vi "Add Item.vi"(7 "Action":T1, 8 "error in (no error)":errorcluster, 11 "Listbox Refs in":T2 {"Section Ref" format="%.0x"}) -> (0 "error out":errorcluster, 3 "Listbox Refs out":T2 {"Section Ref" format="%.0x"})   [LabVIEW 2019, in "FPGA Addon System Explorer.lvlib"]
uses:
  FPGA Addon System Explorer.lvlib
  Types/Listbox Cluster.ctl
  <vilib>/NI VeriStand/Custom Device API/Custom Device Item Ref.ctl
  Types/Channel Type.ctl
  Addon Shared/Types/FG Action.ctl
  <vilib>/NI VeriStand/Custom Device API/Custom Device Channel.ctl
  <vilib>/NI VeriStand/Custom Device API/Custom Device Channel Type.ctl
  Addon Shared/SubVIs/Constants.vi
  <vilib>/NI/NI VeriStand Advanced SysDef API/SysDef API/SysDef.Property.Get.vi
  <vilib>/NI/NI VeriStand Advanced SysDef API/_SubVIs/SysDef.Property.Get.Variant.vi
  <vilib>/NI/NI VeriStand Advanced SysDef API/SysDef API/SysDef.Property.Set.vi
  <vilib>/NI/NI VeriStand Advanced SysDef API/_SubVIs/SysDef.Property.Set.Variant.vi
  <vilib>/NI VeriStand/Custom Device API/Custom Device API.lvlib
  Addon Shared/FPGA Addon Shared.lvlib
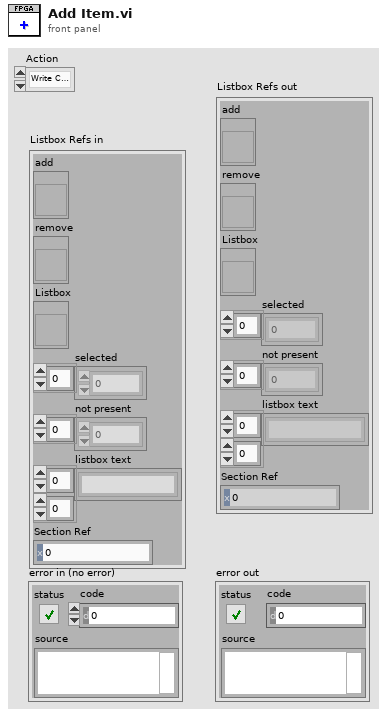
[diagram p1: front panel]
types:
  T1 = typedef "FPGA Addon System Explorer.lvlib/Channel Type.ctl" = enum16{"Write Channel", "Read Channel", "Write Waveform", "Read Waveform"}
  T2 = typedef "FPGA Addon System Explorer.lvlib/Listbox Cluster.ctl" = cluster{"add":refnum<vi>, "remove":refnum<vi>, "Listbox":refnum<vi>, "selected":i32[], "not present":i32[], "listbox text":string[][], "Section Ref":T3}
  T3 = typedef "Custom Device API.lvlib/Custom Device Item Ref.ctl" = u64
  T4 = typedef "FPGA Addon Shared.lvlib/FG Action.ctl" = enum8{"GET", "SET"}
  T5 = typedef "FPGA Addon Shared.lvlib/Register Information.ctl" = cluster{"Name":string, "Data Type":T6, "Default Value":variant}
  T6 = typedef "FPGA Addon Shared.lvlib/Data Type.ctl" = enum8{"<Null>", "I8", "I16", "I32", "I64", "U8", "U16", "U32", "U64", "SGL", "Boolean", "Analog PWM In Settings", "Analog PWM In", "Digital PWM In Settings", "Digital PWM In", "Digital PWM Out", "Sine Out", "FXP+/-24.5", "FXP+/-16.5", "FXP+/-32.8", "FXP+/-64.32", "FXP+/-16.7", "FXP+/-20.5", "FXP+/-27.5", "FXP+/-32.16", "FXP+16.3", "FXP+18.3", "Digital Static In", "Digital Static Out", "Digital Static In Settings", "Digital WSS Out", "Quad Encoder Settings", "Quad Encoder In", "Group"}
  T7 = typedef "Custom Device API.lvlib/Custom Device Channel.ctl" = cluster{"Type":T8, "Units":string, "Default Value":dbl, "Faultable":bool, "Scalable":bool}
  T8 = typedef "Custom Device API.lvlib/Custom Device Channel Type.ctl" = enum16{"Input", "Output"}
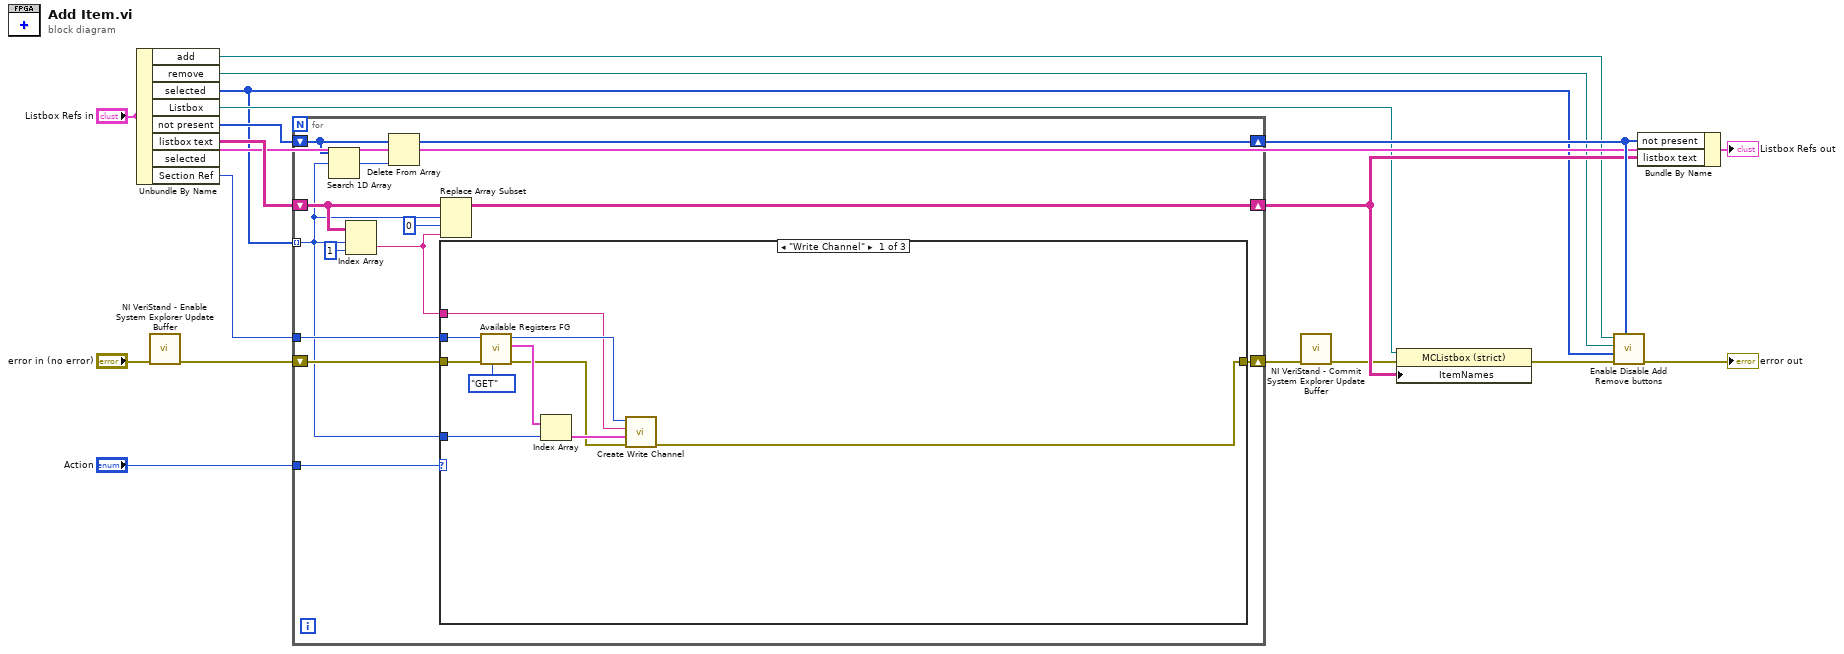
[diagram p0: block diagram]
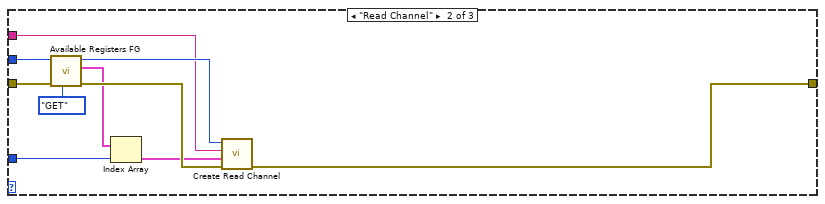
[diagram p2: hidden frame]
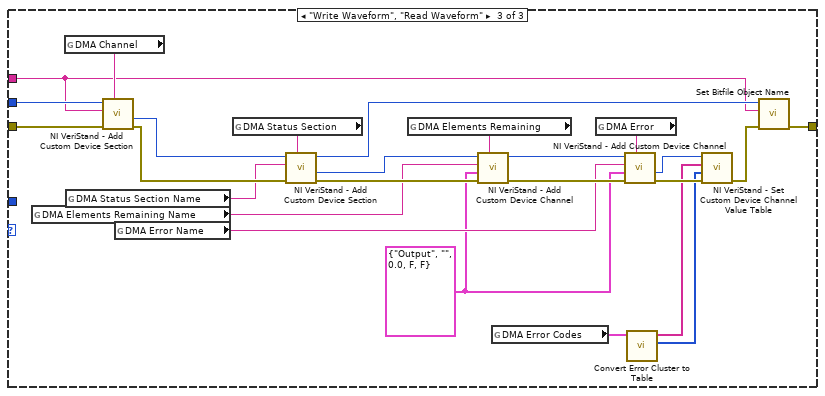
[diagram p3: hidden frame]
diagram:
  n1 = Unbundle By Name("Listbox Refs in") -> ("add"=w10:refnum<vi>, "remove"=w11:refnum<vi>, "selected"=w3:i32[], "Listbox"=w4:refnum<vi>, "not present"=w9:i32[], "listbox text"=w17:string[][], "Section Ref"=w5:T3)  [unwired: 1 out]
  n2 = call <vilib>:"NI VeriStand - Enable System Explorer Update Buffer.vi"("error in (no error)"="error in (no error)") -> ("error out"=w8:errorcluster)  [unwired: 10 in]
  n3 = for {
    tunnel: w5 -> [w30]
    shift-right: [w19] -> w6
    shift-left: w8 -> [w31]
    tunnel: w3 -> [w21] mode=indexing
    shift-right: [w27] -> w15
    shift-left: w17 -> [w28]
    shift-right: [w23] -> w16
    shift-left: w9 -> [w25]
    tunnel: "Action" -> [w22]
    n4 = Search 1D Array(1D array=w25, element=w21) -> (index of element=w24:i32)  [unwired: 1 in]
    n5 = Index Array(array=w28, index (row)=w21, index (col)=1 ("disabled index (col)")) -> (element=w20:string)
    n6 = Delete From Array(array=w25, index=w24) -> (array with subset deleted=w23:i32[])  [unwired: 1 in, 1 out]
    n7 = case shown="\"Write Channel\"" w22 {
      tunnel: w31 -> [w38 w48 w75]
      tunnel: [w34 w51 w53] -> w19
      tunnel: w30 -> [w37 w49 w76]
      tunnel: w20 -> [w32 w42 w52]
      tunnel: w21 -> [w35 w45 _]
      frame "Write Channel" {
        n8 = call "Available Registers FG.vi"("Action"=FG_Action."GET", "error in (no error)"=w38, "Item Ref"=w37) -> ("error out"=w36:errorcluster, "Available Registers"=w40:T5[], "Item Ref out"=w33:T3)  [unwired: 6 in]
        n9 = Index Array(array=w40, index=w35) -> (element=w39:T5)
        n10 = call "Create Write Channel.vi"("error in (no error)"=w36, "Cluster"=w39, "Bitfile Name"=w32, "Item Ref in"=w33) -> ("error out"=w34:errorcluster)  [unwired: 7 in]
      }
      frame "Read Channel" {
        n11 = call "Available Registers FG.vi"("Action"=FG_Action."GET", "error in (no error)"=w48, "Item Ref"=w49) -> ("error out"=w47:errorcluster, "Available Registers"=w46:T5[], "Item Ref out"=w43:T3)  [unwired: 6 in]
        n12 = Index Array(array=w46, index=w45) -> (element=w44:T5)
        n13 = call "Create Read Channel.vi"("error in (no error)"=w47, "Channel"=w44, "Bitfile Name"=w42, "Item Ref in"=w43) -> ("error out"=w51:errorcluster)  [unwired: 7 in]
      }
      frame "Write Waveform", "Read Waveform" {
        w63 = T7 {"Type"=enum."Output", "Units"="", "Default Value"=0.0, "Faultable"=FALSE, "Scalable"=FALSE} ("Channel")
        n14 = global read "Constants.vi" "DMA Elements Remaining Name"() -> (w66:string)
        n15 = global read "Constants.vi" "DMA Channel"() -> (w74:string)
        n16 = global read "Constants.vi" "DMA Status Section Name"() -> (w62:string)
        n17 = call <vilib>:"NI VeriStand - Add Custom Device Section.vi"("GUID (Default Section)"=w74, "error in (no error)"=w75, "Section Name"=w52, "Parent Ref in"=w76) -> ("error out"=w73:errorcluster, "Section Ptr"=w72:T3)  [unwired: 4 in, 2 out]
        n18 = global read "Constants.vi" "DMA Error Name"() -> (w65:string)
        n19 = global read "Constants.vi" "DMA Status Section"() -> (w61:string)
        n20 = call <vilib>:"NI VeriStand - Add Custom Device Section.vi"("GUID (Default Section)"=w61, "error in (no error)"=w73, "Section Name"=w62, "Parent Ref in"=w72) -> ("error out"=w68:errorcluster, "Section Ptr"=w69:T3, "Parent Ref out"=w54:T3)  [unwired: 4 in, 1 out]
        n21 = global read "Constants.vi" "DMA Elements Remaining"() -> (w67:string)
        n22 = call <vilib>:"NI VeriStand - Add Custom Device Channel.vi"("GUID (Default Channel)"=w67, "error in (no error)"=w68, "Channel"=w63, "Channel Name"=w66, "Parent Ref in"=w69) -> ("error out"=w70:errorcluster, "Parent Ref out"=w71:T3)  [unwired: 3 in, 2 out]
        n23 = global read "Constants.vi" "DMA Error Codes"() -> (w60:cluster{"number":i32, "trimmed string":string}[])
        n24 = global read "Constants.vi" "DMA Error"() -> (w64:string)
        n25 = call <vilib>:"NI VeriStand - Add Custom Device Channel.vi"("GUID (Default Channel)"=w64, "error in (no error)"=w70, "Channel"=w63, "Channel Name"=w65, "Parent Ref in"=w71) -> ("error out"=w58:errorcluster, "Channel Ref"=w59:T3)  [unwired: 3 in, 2 out]
        n26 = call "Convert Error Cluster to Table.vi"("Error Codes"=w60) -> ("Code"=w56:i32[], "String"=w57:string[])  [unwired: 9 in]
        n27 = call <vilib>:"NI VeriStand - Set Custom Device Channel Value Table.vi"("error in (no error)"=w58, "Values"=w56, "Names"=w57, "Channel Ref in"=w59) -> ("error out"=w55:errorcluster)  [unwired: 6 in, 1 out]
        n28 = call "Set Bitfile Object Name.vi"("error in (no error)"=w55, "Name"=w52, "Channel Ref"=w54) -> ("error out"=w53:errorcluster)  [unwired: 8 in]
      }
    }
    n29 = Replace Array Subset(array=w28, new element=w20, index (row)=w21, index (col)=0 ("disabled index (col)")) -> (w27:string[][])
  }
  n30 = call <vilib>:"NI VeriStand - Commit System Explorer Update Buffer.vi"("error in (no error)"=w6) -> ("error out"=w13:errorcluster)  [unwired: 10 in]
  n31 = property class="MCListbox (strict)"(reference=w4, error in=w13, "ItemNames"=w15) -> (error out=w12:errorcluster)  [unwired: 1 out]
  n32 = call "Enable Disable Add Remove buttons.vi"("not present item indexes"=w16, "error in (no error)"=w12, "selected items"=w3, "remove button"=w11, "add button"=w10) -> ("error out"=→"error out":errorcluster)  [unwired: 6 in]
  n33 = Bundle By Name(cluster="Listbox Refs in", "not present"=w16, "listbox text"=w15) -> (→"Listbox Refs out":T2)
